vi "[ce] LM Fit - formula evaluator.vi"(5 "formula params":T2, 7 "VC Handle":T1=-1, 8 "error in":errorcluster, 9 "action":enum16{"init", "close", "calculate"}(ring)=enum."calculate", 10 "X (for init only)":dbl[](array[numeric]) format="%.2f", 11 "coef values":dbl[](array[numeric]) format="%.2f") -> (0 "error out":errorcluster, 2 "calc result":dbl[](array[numeric]) format="%.2f", 3 "coef values out":dbl[](array[numeric]) format="%.2f")   [LabVIEW 2021]
doc: "::: CalcExpress Toolkit :::\nCopyright (c) 2000-2026 Konstantin Shifershteyn. All rights reserved."
uses:
  [ce] LM Fit - model description.ctl
  cetypes.llb/VarMan Variable Context Handle.ctl
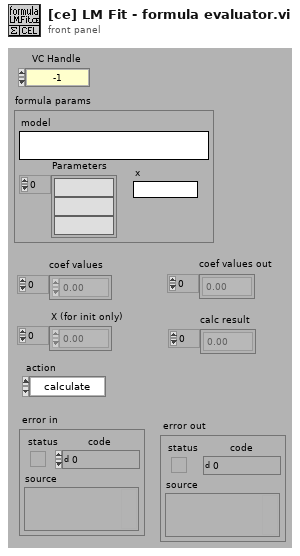
[diagram p1: front panel]
types:
  T1 = typedef "VarMan Variable Context Handle.ctl" = i32
  T2 = typedef "[ce] LM Fit - model description.ctl" = cluster{"model":string, "Parameters":string[], "x":string}
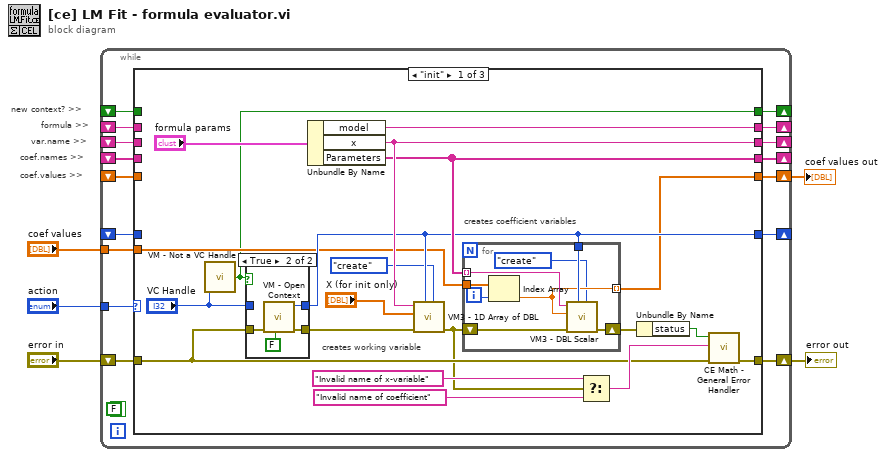
[diagram p0: block diagram]
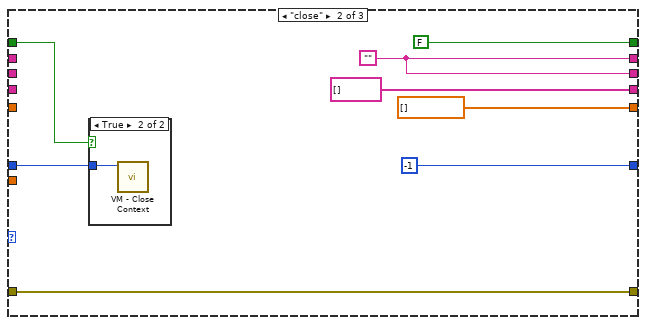
[diagram p3: hidden frame]
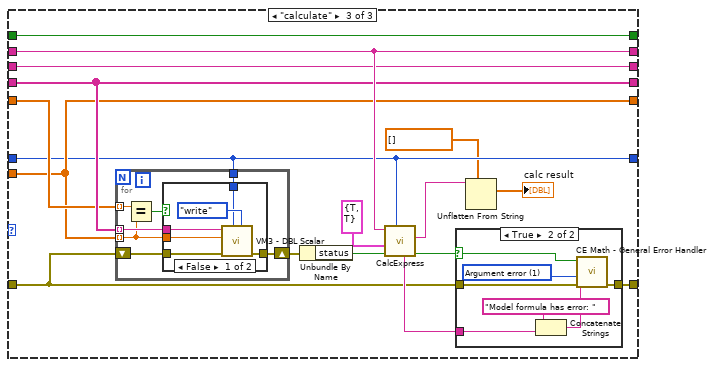
[diagram p5: hidden frame]
diagram:
  # "new context? >>"
  # "coef.values >>"
  # "coef.names >>"
  # "var.name >>"
  # "formula >>"
  n1 = while {
    shift-left: _ -> [w9]
    shift-right: [w10] -> w1
    shift-left: "error in" -> [w11]
    shift-right: [w12] -> w3
    tunnel: "coef values" -> [w13]
    tunnel: "action" -> [w18]
    shift-left: _ -> [w16]
    shift-right: [w19] -> _
    shift-left: _ -> [w14]
    shift-right: [w20] -> _
    shift-left: _ -> [w17]
    shift-right: [w21] -> _
    shift-left: _ -> [w15]
    shift-right: [w22] -> _
    shift-right: [w7] -> _
    shift-left: _ -> [w6]
    stop <- FALSE continue-if-true
    n2 = case shown="\"init\"" w18 {
      tunnel: [w42 w63 w81] -> w22
      tunnel: [w37 T1 -1 ("VC Handle out") w76] -> w21
      tunnel: [w41 string[] [] ("coef.names") w80] -> w20
      tunnel: [w38 w63 w82] -> w19
      tunnel: w17 -> [_ w64 w76]
      tunnel: w16 -> [_ _ w82]
      tunnel: w15 -> [_ _ w81]
      tunnel: w14 -> [_ _ w80]
      tunnel: w13 -> [w32 _ w78]
      tunnel: [w33 w60 w71] -> w12
      tunnel: w11 -> [w27 w60 w67]
      tunnel: [w31 dbl[] [] ("coefs in") w78] -> w10
      tunnel: w9 -> [_ _ w79]
      tunnel: [w28 FALSE ("Not a VC Handle") w68] -> w7
      tunnel: w6 -> [_ w58 w68]
      frame "init" {
        # "creates working variable"
        # "creates coefficient variables"
        n3 = call "VM - Not a VC Handle.vi"("VC Handle"="VC Handle") -> ("Not a VC Handle"=w28:bool)  [unwired: 1 in]
        n4 = case shown="True" w28 {
          tunnel: [w44 w48] -> w26
          tunnel: [w43 w47] -> w37
          tunnel: w27 -> [w44 w46]
          tunnel: "VC Handle" -> [w43 _]
          frame False {
          }
          frame True {
            n5 = call "VM - Open Context.vi"("close loose contexts (F)"=FALSE ("close loose contexts (T)"), "error in"=w46) -> ("error out"=w48:errorcluster, "VC Handle out"=w47:T1)  [unwired: 7 in, 1 out]
          }
        }
        n6 = Unbundle By Name("formula params") -> ("model"=w38:string, "x"=w42:string, "Parameters"=w41:string[])
        n7 = call "VM3 - 1D Array of DBL.vi"("cmd (read)"=enum16{"create", "destroy", "write", "read"}."create", "VC Handle"=w37, "error in"=w26, "value in"="X (for init only)", "name_spec"=w42) -> ("error out"=w25:errorcluster)  [unwired: 3 in, 3 out]
        n8 = for {
          tunnel: w41 -> [w56] mode=indexing
          shift-right: [w54] -> w30
          shift-left: w25 -> [w55]
          tunnel: w37 -> [w53]
          tunnel: w32 -> [w51]
          tunnel: [w50] -> w31 mode=indexing
          i -> [w52]
          n9 = Index Array(array=w51, index=w52) -> (element=w50:dbl)
          n10 = call "VM3 - DBL Scalar.vi"("cmd (read)"=enum16{"create", "destroy", "write", "read"}."create", "VC Handle"=w53, "error in"=w55, "value in"=w50, "name_spec"=w56) -> ("error out"=w54:errorcluster)  [unwired: 3 in, 3 out]
        }
        n11 = Select(t="Invalid name of x-variable" ("Reason"), s=w25, f="Invalid name of coefficient" ("Reason")) -> (s? t:f=w34:string)
        n12 = Unbundle By Name(w30) -> ("status"=w23:bool)
        n13 = call "CE Math - General Error Handler.vi"("error before"=w27, "message"=w34, "error? (T)"=w23) -> ("error out"=w33:errorcluster)  [unwired: 5 in, 1 out]
      }
      frame "close" {
        w63 = ""
        n14 = case shown="True" w58 {
          tunnel: w64 -> [_ w65]
          frame False {
          }
          frame True {
            n15 = call "VM - Close Context.vi"("VC Handle"=w65) -> ()  [unwired: 9 in, 2 out]
          }
        }
      }
      frame "calculate" {
        n16 = for {
          tunnel: w80 -> [w97] mode=indexing
          tunnel: w78 -> [w93] mode=indexing
          shift-right: [w96] -> w77
          shift-left: w67 -> [w95]
          tunnel: w76 -> [w94]
          tunnel: w79 -> [w91] mode=indexing
          n17 = Equal?(x=w91, y=w93) -> (x = y?=w92:bool)
          n18 = case shown="False" w92 {
            tunnel: w97 -> [w103 _]
            tunnel: w93 -> [w102 _]
            tunnel: [w101 w104] -> w96
            tunnel: w95 -> [w99 w104]
            tunnel: w94 -> [w98 _]
            frame False {
              n19 = call "VM3 - DBL Scalar.vi"("cmd (read)"=enum16{"create", "destroy", "write", "read"}."write", "VC Handle"=w98, "error in"=w99, "value in"=w102, "name_spec"=w103) -> ("error out"=w101:errorcluster)  [unwired: 3 in, 3 out]
            }
            frame True {
            }
          }
        }
        n20 = Unbundle By Name(w77) -> ("status"=w66:bool)
        n21 = call "CalcExpress.vi"("VC Handle"=w76, "error in"=w66, "params"=cluster{"autoVar":bool, "enCpx":bool} {"autoVar"=TRUE, "enCpx"=TRUE}, "expression"=w82) -> ("error out"=w70:bool, "string value"=w74:string, "error description"=w69:string)  [unwired: 3 in, 2 out]
        n22 = case shown="True" w70 {
          selector: w70 -> [_ w84]
          tunnel: [w83 w88] -> w71
          tunnel: w69 -> [_ w87]
          tunnel: w67 -> [w83 w86]
          frame False {
          }
          frame True {
            w85 = u16 1 items=["No error", "Argument error", "Memory is full", "Out of zone", "End of file", "File already open", "Generic file I/O error", "File not found", "File permission error", "Disk is full", "Duplicate path", "Too many files open", "System feature not enabled", "Resource file not found", "Cannot add resource", "Resource not found", "Image not found", "Image memory error", "Pen does not exist", "Config type invalid", "Config token not found", "Config parse error", "Config memory error", "Bad external code format", "Bad external code offset", "External code not present", "Null window", "Destroy window error", "Null menu", "Print aborted", "Bad print record", "Print driver error", "Windows error during printing", "Memory error during printing", "Print dialog error", "Generic print error", "Invalid device refnum", "Device not found", "Device parameter error", "Device unit error", "Cannot open device", "Device call aborted", "Generic error", "Cancelled by user", "Object ID too low", "Object ID too high", "Object not in heap", "Unknown heap", "Unknown object (invalid DefProc)", "Unknown object (DefProc not in table)", "Message out of range", "Invalid (null) method", "Unknown message", "Manager call not supported", "Bad address", "Network operation in progress", "Network operation timed out", "Connection is busy", "Network attribute not supported", "Network error", "Address in use", "System out of memory", "Connection aborted", "Connection refused", "Not connected", "Already connected", "Connection closed", "Initialization error (interapplication manager)", "Bad occurrence", "Wait on unbound occurrence handler", "Occurrence queue overflow", "Datalog type conflict", "Unused", "Unrecognized type (interapplication manager)", "Memory corrupt", "Failed to make temporary DLL", "Old CIN version", "Drag socket not found", "Failed to load drop-object", "Failed to register OLE object", "Failed to release OLE object", "Format specifier type mismatch", "Unknown format specifier", "Too few format specifiers", "Too many format specifiers", "Scan failed", "Newer CIN version", "OLE Convert", "Runtime menu error", "Password tampered", "Unknown error code"]
            n23 = Concatenate Strings("Model formula has error: ", w87) -> (w90:string)
            n24 = call "CE Math - General Error Handler.vi"("error before"=w86, "error code"=w85, "message"=w90, "error? (T)"=w84) -> ("error out"=w88:errorcluster)  [unwired: 4 in, 1 out]
          }
        }
        n25 = Unflatten From String(type=dbl[] [] ("coefficient values"), binary string=w74) -> (value=→"calc result":dbl[])  [unwired: 3 in, 2 out]
      }
    }
  }
  "error out" <- w3
  "coef values out" <- w1
